vi "[ex ce] History Speed (CSE & DBL array).vi"() -> ()   [LabVIEW 2021]
doc: "<B>Run speed example</B>\n\nThe VI demonstrates how a variable history affects execution speed.\n\n::: CalcExpress Toolkit :::\nCopyright (c) 2000-2026 Konstantin Shifershteyn. All rights reserved."
panel:
  out "value out":dbl[](array[numeric]) format="%#_9g"
  in  "reverse order":bool=TRUE caption="Read history in reversed order"
  out "Historic values":cluster{"Array":dbl[]}[](array[cluster]) {"Array" format="%#_9g"}
  out "read history, ms":u32
  out "speed ratio":dbl format="%.2f"
  out "with history, ms":u32
  out "without history, ms":u32
  in  "history length":i32=1000
  in  "script":string="/*\n'vec' variable is 1D array, it's created in the script. A value assigned to it is an array of 100 elements in the range from 0 up to 99 with the step of 1.\n*/\n\nvec = nvecins(0, 1000, 1);\n\n/*\n'x' variable is 1D array, it's created on the VI Block Diagram. The variable is updated 10000 times in the loop.\n*/\n\nfor (i=0; i<100000; i+=1) {\n  x = vec + i;\n}"
  # "1) history length has large sense for memory use but it does not influence a lot on CPU use.\n2) size of array ('x' variable here) influences very much on both memory and CPU use."
  # "execution time"
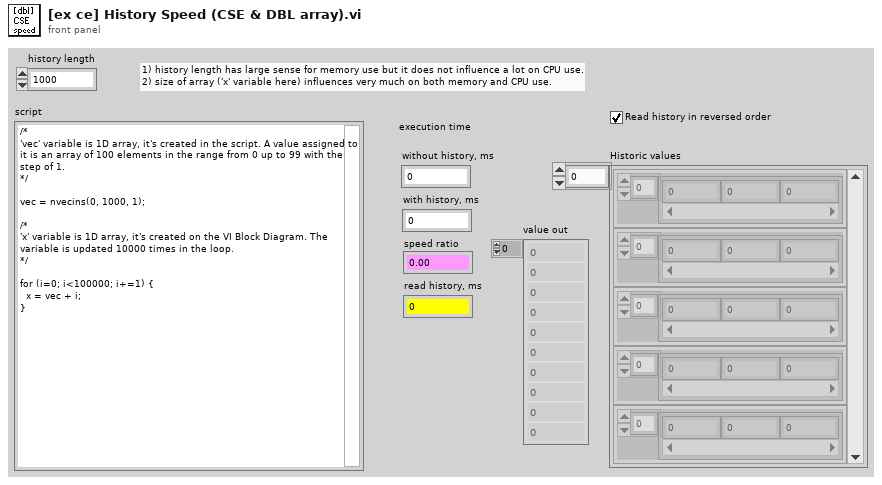
[diagram p1: front panel]
types:
  T1 = enum16{"create", "destroy", "set value", "get value"}
  T2 = enum32{"nop", "create", "destroy", "reset", "get info", "config"}
  T3 = typedef "VarMan Variable Context Handle.ctl" = i32
  T4 = typedef "CSE Instance RefNum.ctl" = refnum<k1>
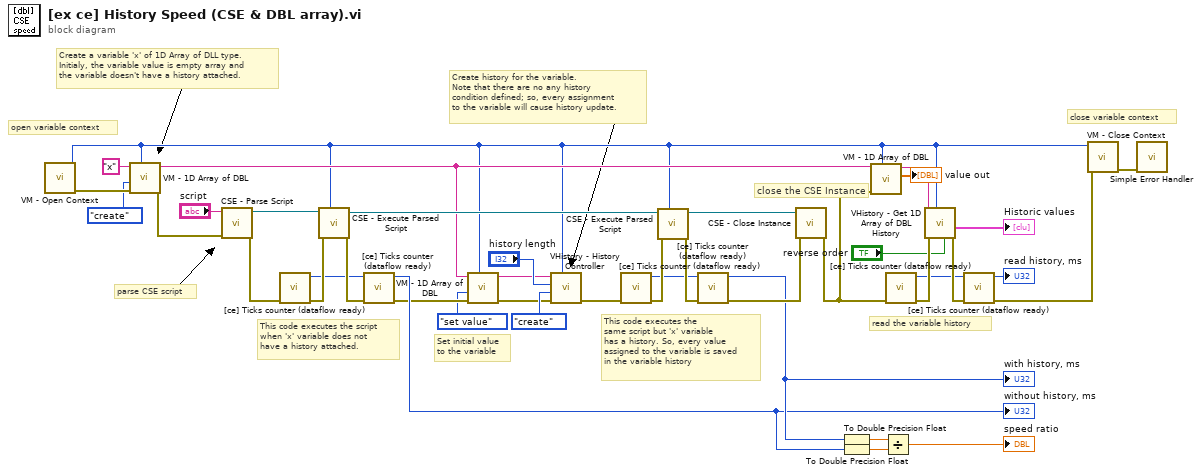
[diagram p0: block diagram]
diagram:
  # "parse CSE script"
  # "Create history for the variable.\nNote that there are no any history\ncondition defined; so, every assignment\nto the variable will cause history update."
  # "Create a variable 'x' of 1D Array of DLL type.\nInitialy, the variable value is empty array and\nthe variable doesn't have a history attached."
  # "Set initial value\nto the variable"
  # "close variable context"
  # "read the variable history"
  # "close the CSE Instance"
  # "open variable context"
  # "This code executes the\nsame script but 'x' variable\nhas a history. So, every value\nassigned to the variable is saved\nin the variable history"
  # "This code executes the script\nwhen 'x' variable does not\nhave a history attached."
  n1 = call "VM - Open Context.vi"() -> ("error out"=w39:errorcluster, "VC Handle out"=w4:T3)  [unwired: 9 in, 1 out]
  n2 = call "VM - 1D Array of DBL.vi"("VC Handle"=w4, "error in"=w39, "cmd"=T1."create", "name_spec"="x" ("name")) -> ("error out"=w25:errorcluster, "dup name_spec"=w5:string)  [unwired: 2 in, 4 out]
  n3 = call "CSE - Parse Script.vi"("error in"=w25, "Script"="script") -> ("error out"=w35:errorcluster, "CSE RefNum"=w28:T4)  [unwired: 5 in, 3 out]
  n4 = call "[ce] Ticks counter (dataflow ready).vi"("error in"=w35) -> ("error out"=w34:errorcluster, "ticks (current-input)"=w24:u32)  [unwired: 4 in, 3 out]
  n5 = call "CSE - Execute Parsed Script.vi"("VC Handle"=w4, "error in"=w34, "CSE RefNum"=w28) -> ("error out"=w33:errorcluster, "dup CSE RefNum"=w29:T4)  [unwired: 4 in, 3 out]
  n6 = call "[ce] Ticks counter (dataflow ready).vi"("error in"=w33, "ticks in"=w24) -> ("error out"=w9:errorcluster, "ticks (current-input)"=w21:u32)  [unwired: 3 in, 3 out]
  "without history, ms" <- w21
  n7 = call "VM - 1D Array of DBL.vi"("VC Handle"=w4, "error in"=w9, "cmd"=T1."set value", "name_spec"=w5) -> ("error out"=w8:errorcluster, "dup name_spec"=w7:string)  [unwired: 2 in, 4 out]
  n8 = call "VHistory - History Controller.vi"("VC Handle"=w4, "error in"=w8, "cmd (nop:default)"=T2."create", "history length"="history length", "name_spec"=w7) -> ("error out"=w30:errorcluster)  [unwired: 3 in, 3 out]
  n9 = call "[ce] Ticks counter (dataflow ready).vi"("error in"=w30) -> ("error out"=w31:errorcluster, "ticks (current-input)"=w23:u32)  [unwired: 4 in, 3 out]
  n10 = call "CSE - Execute Parsed Script.vi"("VC Handle"=w4, "error in"=w31, "CSE RefNum"=w29) -> ("error out"=w32:errorcluster, "dup CSE RefNum"=w27:T4)  [unwired: 4 in, 3 out]
  n11 = call "[ce] Ticks counter (dataflow ready).vi"("error in"=w32, "ticks in"=w23) -> ("error out"=w26:errorcluster, "ticks (current-input)"=w22:u32)  [unwired: 3 in, 3 out]
  "with history, ms" <- w22
  n12 = call "CSE - Close Instance.vi"("error in"=w26, "CSE RefNum"=w27) -> ("error out"=w2:errorcluster)  [unwired: 5 in, 2 out]
  n13 = To Double Precision Float(number=w22) -> (double precision float=w13:dbl)
  n14 = To Double Precision Float(number=w21) -> (double precision float=w12:dbl)
  n15 = call "VM - 1D Array of DBL.vi"("VC Handle"=w4, "error in"=w2, "name_spec"=w5) -> ("value out"=→"value out":dbl[], "dup name_spec"=w3:string)  [unwired: 3 in, 4 out]
  n16 = Divide(x=w13, y=w12) -> (x/y=→"speed ratio":dbl)
  n17 = call "[ce] Ticks counter (dataflow ready).vi"("error in"=w2) -> ("error out"=w19:errorcluster, "ticks (current-input)"=w16:u32)  [unwired: 4 in, 3 out]
  n18 = call "VHistory - Get 1D Array of DBL History.vi"("reverse order (T)"="reverse order", "VC Handle"=w4, "error in"=w19, "name_spec"=w3) -> ("error out"=w18:errorcluster, "history"=→"Historic values":cluster{"data":dbl[]}[])  [unwired: 3 in, 3 out]
  n19 = call "[ce] Ticks counter (dataflow ready).vi"("error in"=w18, "ticks in"=w16) -> ("error out"=w17:errorcluster, "ticks (current-input)"=→"read history, ms":u32)  [unwired: 3 in, 3 out]
  n20 = call "VM - Close Context.vi"("error in"=w17, "VC Handle"=w4) -> ("error out"=w11:errorcluster)  [unwired: 8 in, 1 out]
  n21 = call <vilib>:"Simple Error Handler.vi"("error in (no error)"=w11) -> ()  [unwired: 4 in, 5 out]
